vi "Send Measurement.vi"(8 "error in (no error)":errorcluster, 10 "Data":dbl[](array[numeric]), 11 "TCP Network Connection in":refnum<k5>) -> (0 "error out":errorcluster, 3 "TCP Network Connection out":refnum<k5>)   [LabVIEW 2026]
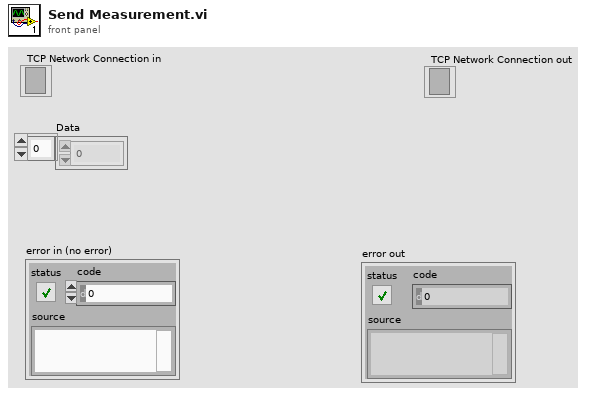
[diagram p1: front panel]
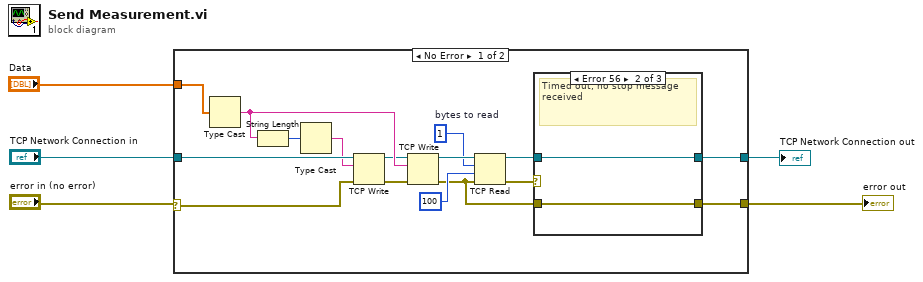
[diagram p0: block diagram]
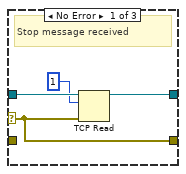
[diagram p2: hidden frame]
diagram:
  n1 = case shown="No Error" "error in (no error)" {
    selector: "error in (no error)" -> [w6 w31]
    tunnel: "Data" -> [w21 _]
    tunnel: [w20 w31] -> w4
    tunnel: "TCP Network Connection in" -> [w19 w30]
    tunnel: [w7 w30] -> w2
    frame No Error {
      w13 = 1  # bytes to read
      n2 = Type Cast(x=w21) -> (*(type *) &x=w12:string)  [unwired: 1 out]
      n3 = String Length(string=w12) -> (length=w10:i32)
      n4 = Type Cast(x=w10) -> (*(type *) &x=w11:string)  [unwired: 1 out]
      n5 = TCP Write(connection ID=w19, data in=w11, error in (no error)=w6) -> (connection ID out=w8:refnum<k5>, error out=w9:errorcluster)  [unwired: 2 out]
      n6 = TCP Write(connection ID=w8, data in=w12, error in (no error)=w9) -> (connection ID out=w14:refnum<k5>, error out=w16:errorcluster)  [unwired: 2 out]
      n7 = TCP Read(connection ID=w14, bytes to read=w13, error in (no error)=w16, 9:100 ("milliseconds to wait")) -> (connection ID out=w18:refnum<k5>, error out=w15:errorcluster)  [unwired: 2 out]
      n8 = case shown="Error 56" w15 {
        selector: w15 -> [w23 _ w29]
        tunnel: [w23 w27 w29] -> w20
        tunnel: w16 -> [_ w27 _]
        tunnel: w18 -> [w25 w26 w28]
        tunnel: [w24 w26 w28] -> w7
        frame No Error {
          # "Stop message received"
          n9 = TCP Read(connection ID=w25, bytes to read=1, error in (no error)=w23) -> (connection ID out=w24:refnum<k5>)  [unwired: 1 in, 3 out]
        }
        frame Error {
          # "Timed out; no stop message received"
        }
        frame Default {
          # "Some other error occurred"
        }
      }
    }
    frame Error {
    }
  }
  "error out" <- w4
  "TCP Network Connection out" <- w2
